vi "test_PhotonPoseEstimator_ClosestToRefPose.vi"(8 "error in (no error)":errorcluster) -> (0 "error out":errorcluster, 3 "Test Passed":bool)   [LabVIEW 2019]
uses:
  <vilib>/Rock Robotics/WPI/ThirdParty/PhotonVisionLib/TypeDef/PhotonEstimatedRobotPoseType.ctl
  <vilib>/Rock Robotics/WPI/ThirdParty/JAS_Junk/TrajLib/TypeDef/POSE3D.ctl
  <vilib>/Rock Robotics/WPI/ThirdParty/JAS_Junk/TrajLib/TypeDef/TRANSLATION3D.ctl
  <vilib>/Rock Robotics/WPI/ThirdParty/JAS_Junk/TrajLib/TypeDef/ROTATION3D.ctl
  <vilib>/Rock Robotics/WPI/ThirdParty/JAS_Junk/TrajLib/TypeDef/QUATERNION.ctl
  <vilib>/Rock Robotics/WPI/ThirdParty/PhotonVisionLib/TypeDef/PhotonTrackedTargetType.ctl
  <vilib>/Rock Robotics/WPI/ThirdParty/PhotonVisionLib/TypeDef/TargetCornerType.ctl
  <vilib>/Rock Robotics/WPI/ThirdParty/JAS_Junk/TrajLib/TypeDef/TRANSFORM3D.ctl
  <vilib>/Rock Robotics/WPI/ThirdParty/PhotonVisionLib/Enum/PhotonPoseStrategy_ENUM.ctl
  <vilib>/Rock Robotics/WPI/ThirdParty/JAS_Junk/TrajLib/VI/Quaternion_New.vi
  <vilib>/Rock Robotics/WPI/ThirdParty/PhotonVisionLib/SubVI/PhotonTargetModel_New_AprilTag36H11.vi
  <vilib>/Rock Robotics/WPI/ThirdParty/JAS_Junk/TrajLib/VI/TimeInterpRotation2d_New.vi
  <vilib>/Rock Robotics/WPI/ThirdParty/PhotonVisionLib/SubVI/PhotonPoseEstimator_Update_All.vi
  <vilib>/Rock Robotics/WPI/ThirdParty/PhotonVisionLib/SubVI/PhotonTargetModel_New_RectPlanar.vi
  <vilib>/Rock Robotics/WPI/ThirdParty/JAS_Junk/TrajLib/Conv_Inches_Meters.vi
  <vilib>/Rock Robotics/WPI/ThirdParty/PhotonVisionLib/SubVI/PhotonPoseEstimator_SetLastPose.vi
  <vilib>/Rock Robotics/WPI/ThirdParty/PhotonVisionLib/SubVI/PhotonPoseEstimator_GetEmptyPose.vi
  <vilib>/Rock Robotics/WPI/ThirdParty/PhotonVisionLib/SubVI/PhotonPoseEstimator_EstimateLowestAmbiguityPose.vi
  <vilib>/Rock Robotics/WPI/ThirdParty/PhotonVisionLib/SubVI/PhotonPoseEstimator_EstimateClosestToCameraHeightPose.vi
  <vilib>/Rock Robotics/WPI/ThirdParty/PhotonVisionLib/SubVI/PhotonPoseEstimator_EstimateClosestToReferencePose.vi
  <vilib>/Rock Robotics/WPI/ThirdParty/PhotonVisionLib/SubVI/PhotonPoseEstimator_GetReferencePose.vi
  <vilib>/Rock Robotics/WPI/ThirdParty/PhotonVisionLib/SubVI/PhotonPoseEstimator_GetLastPose.vi
  <vilib>/Rock Robotics/WPI/ThirdParty/PhotonVisionLib/SubVI/PhotonPoseEstimator_EstimateClosestToLastPose.vi
  <vilib>/Rock Robotics/WPI/ThirdParty/PhotonVisionLib/SubVI/PhotonPoseEstimator_EstimateAverageBestTargetsPose.vi
  <vilib>/Rock Robotics/WPI/ThirdParty/PhotonVisionLib/SubVI/PhotonPoseEstimator_EstimateMultiTagOnCoprocPose.vi
  <vilib>/Rock Robotics/WPI/ThirdParty/PhotonVisionLib/SubVI/PhotonPoseEstimator_EstimatePnpDistanceTrigSolvePose.vi
  <vilib>/Rock Robotics/WPI/ThirdParty/PhotonVisionLib/SubVI/PhotonPoseEstimator_Strategy_constrainedPnpStrategy.vi
  <vilib>/Rock Robotics/WPI/ThirdParty/PhotonVisionLib/SubVI/PhotonPipelineResult_GetTimeStampSecs.vi
  <vilib>/Rock Robotics/WPI/ThirdParty/PhotonVisionLib/SubVI/PhotonTargetModel_New.vi
  <vilib>/Rock Robotics/WPI/ThirdParty/JAS_Junk/TrajLib/VI/Rotation3d_Create_AxisAngle.vi
  <vilib>/Rock Robotics/WPI/ThirdParty/JAS_Junk/TrajLib/VI/Pose3d_New.vi
  <vilib>/Rock Robotics/WPI/ThirdParty/PhotonVisionLib/SubVI/PhotonPipelineResult_HasTargets.vi
  <vilib>/Rock Robotics/WPI/ThirdParty/PhotonVisionLib/SubVI/PhotonPipelineResult_GetTargets.vi
  <vilib>/Rock Robotics/WPI/ThirdParty/PhotonVisionLib/SubVI/PhotonTrackedTarget_GetPoseAmbiguity.vi
  <vilib>/Rock Robotics/WPI/ThirdParty/PhotonVisionLib/SubVI/PhotonTrackedTarget_GetFiducialId.vi
  <vilib>/Rock Robotics/WPI/ThirdParty/PhotonVisionLib/SubVI/PhotonPoseEstimator_GetFieldTags.vi
  <vilib>/Rock Robotics/WPI/ThirdParty/JAS_Junk/TrajLib/VI/AprilTagFieldLayout_GetTagPose.vi
  <vilib>/Rock Robotics/WPI/ThirdParty/JAS_Junk/TrajLib/VI/Pose3d_TransformBy.vi
  <vilib>/Rock Robotics/WPI/ThirdParty/PhotonVisionLib/SubVI/PhotonTrackedTarget_GetBestCameraToTarget.vi
  <vilib>/Rock Robotics/WPI/ThirdParty/JAS_Junk/TrajLib/VI/Transform3d_Inverse.vi
  <vilib>/Rock Robotics/WPI/ThirdParty/PhotonVisionLib/SubVI/PhotonPoseEstimator_GetRobotToCameraTransform.vi
  <vilib>/Rock Robotics/WPI/ThirdParty/PhotonVisionLib/SubVI/PhotonPoseEstimator_GetHighestAmbiguity.vi
  <vilib>/Rock Robotics/WPI/ThirdParty/PhotonVisionLib/SubVI/PhotonEstimatedRobotPose_New.vi
  <vilib>/Rock Robotics/WPI/ThirdParty/PhotonVisionLib/SubVI/PhotonPoseEstimator_Strategy_closestToCameraHeight_calc.vi
  <vilib>/Rock Robotics/WPI/ThirdParty/PhotonVisionLib/SubVI/PhotonTrackedTarget_GetAltCameraToTarget.vi
  <vilib>/Rock Robotics/WPI/ThirdParty/PhotonVisionLib/SubVI/PhotonPoseEstimator_Strategy_closestToReferencePose_calc.vi
  <vilib>/Rock Robotics/WPI/ThirdParty/PhotonVisionLib/SubVI/PhotonPoseEstimator_Strategy_averageBestTargets_calc.vi
  <vilib>/Rock Robotics/WPI/ThirdParty/JAS_Junk/TrajLib/VI/Rotation3d_Plus.vi
  <vilib>/Rock Robotics/WPI/ThirdParty/JAS_Junk/TrajLib/VI/Translation3d_Plus.vi
  <vilib>/Rock Robotics/WPI/ThirdParty/JAS_Junk/TrajLib/VI/Translation3d_Times.vi
  <vilib>/Rock Robotics/WPI/ThirdParty/JAS_Junk/TrajLib/VI/Rotation3d_Times.vi
  <vilib>/Rock Robotics/WPI/ThirdParty/JAS_Junk/TrajLib/VI/Rotation3d_Create_Default.vi
  <vilib>/Rock Robotics/WPI/ThirdParty/JAS_Junk/TrajLib/VI/Translation3d_Create_Default.vi
  <vilib>/Rock Robotics/WPI/ThirdParty/JAS_Junk/TrajLib/VI/Pose3d_New_Default.vi
  <vilib>/Rock Robotics/WPI/ThirdParty/JAS_Junk/TrajLib/VI/Pose3d_Plus.vi
  <vilib>/Rock Robotics/WPI/ThirdParty/JAS_Junk/TrajLib/VI/Pose3d_RelativeTo.vi
  <vilib>/Rock Robotics/WPI/ThirdParty/JAS_Junk/TrajLib/VI/AprilTagFieldLayout_GetOriginPosition.vi
  <vilib>/Rock Robotics/WPI/ThirdParty/PhotonVisionLib/SubVI/PhotonPipelineResult_GetMultiTagResult.vi
  <vilib>/Rock Robotics/WPI/ThirdParty/PhotonVisionLib/SubVI/PhotonPipelineResult_GetBestTarget.vi
  <vilib>/Rock Robotics/WPI/ThirdParty/PhotonVisionLib/SubVI/PhotonTrackedTarget_GetPitch.vi
  <vilib>/Rock Robotics/WPI/ThirdParty/PhotonVisionLib/SubVI/PhotonTrackedTarget_GetYaw.vi
  <vilib>/Rock Robotics/WPI/ThirdParty/JAS_Junk/TrajLib/Units_DegreesToRadians.vi
  <vilib>/Rock Robotics/WPI/ThirdParty/JAS_Junk/TrajLib/VI/Transform3d_GetTranslation3d.vi
  <vilib>/Rock Robotics/WPI/ThirdParty/JAS_Junk/TrajLib/VI/Translation3d_GetNorm.vi
  <vilib>/Rock Robotics/WPI/ThirdParty/JAS_Junk/TrajLib/VI/Translation3d_Create_DistAng.vi
  <vilib>/Rock Robotics/WPI/ThirdParty/JAS_Junk/TrajLib/VI/Translation3d_RotateBy.vi
  <vilib>/Rock Robotics/WPI/ThirdParty/JAS_Junk/TrajLib/VI/Translation3d_ToTranslation2d.vi
  <vilib>/Rock Robotics/WPI/ThirdParty/JAS_Junk/TrajLib/Translation2d_RotateBy.vi
  <vilib>/Rock Robotics/WPI/ThirdParty/JAS_Junk/TrajLib/VI/Transform3d_GetRotation3d.vi
  <vilib>/Rock Robotics/WPI/ThirdParty/JAS_Junk/TrajLib/VI/Pose3d_ToPose2d.vi
  <vilib>/Rock Robotics/WPI/ThirdParty/JAS_Junk/TrajLib/Pose2d_getTranslation.vi
  <vilib>/Rock Robotics/WPI/ThirdParty/JAS_Junk/TrajLib/Translation2d_Plus.vi
  <vilib>/Rock Robotics/WPI/ThirdParty/JAS_Junk/TrajLib/Translation2d_UnaryMinus.vi
  <vilib>/Rock Robotics/WPI/ThirdParty/JAS_Junk/TrajLib/Pose2d_New_TRRO.vi
  <vilib>/Rock Robotics/WPI/ThirdParty/JAS_Junk/TrajLib/VI/Pose3d_New_Pose2d.vi
  <vilib>/Rock Robotics/WPI/ThirdParty/JAS_Junk/TrajLib/VI/TimeInterpRotation2d_GetSample.vi
  <vilib>/Rock Robotics/WPI/ThirdParty/PhotonVisionLib/SubVI/PhotonPoseEstimator_GetHeadingBuffer.vi
  <vilib>/Rock Robotics/WPI/ThirdParty/JAS_Junk/TrajLib/VI/Vector_Norm.vi
  <vilib>/Rock Robotics/WPI/ThirdParty/JAS_Junk/TrajLib/VecBuilder_ArrayBy1Fill.vi
  <vilib>/Rock Robotics/WPI/ThirdParty/JAS_Junk/TrajLib/VI/AprilTag_GetAll.vi
  <vilib>/Rock Robotics/WPI/ThirdParty/JAS_Junk/TrajLib/VI/Pose3d_getTranslation3d.vi
  <vilib>/Rock Robotics/WPI/ThirdParty/JAS_Junk/TrajLib/VI/Pose3d_getRotation3d.vi
  <vilib>/Rock Robotics/WPI/ThirdParty/JAS_Junk/TrajLib/VI/Rotation3d_ToRotation2d.vi
  <vilib>/Rock Robotics/WPI/ThirdParty/JAS_Junk/TrajLib/Transform2d_Create_TransRot.vi
  <vilib>/Rock Robotics/WPI/ThirdParty/JAS_Junk/TrajLib/VI/Rotation3d_UnaryMinus.vi
  <vilib>/Rock Robotics/WPI/ThirdParty/JAS_Junk/TrajLib/VI/Translation3d_UnaryMinus.vi
  <vilib>/Rock Robotics/WPI/ThirdParty/JAS_Junk/TrajLib/VI/Transform3d_GetXYZ.vi
  <vilib>/Rock Robotics/WPI/ThirdParty/JAS_Junk/TrajLib/VI/Pose3d_getXYZ.vi
  <vilib>/Rock Robotics/WPI/ThirdParty/PhotonVisionLib/SubVI/PhotonPoseEstimator_CalcDifference.vi
  <vilib>/Rock Robotics/WPI/ThirdParty/JAS_Junk/TrajLib/VI/Rotation3d_RotateBy.vi
  <vilib>/Rock Robotics/WPI/ThirdParty/JAS_Junk/TrajLib/VI/Translation3d_GetXYZ.vi
  <vilib>/Rock Robotics/WPI/ThirdParty/JAS_Junk/TrajLib/VI/Rotation3d_GetQuaterion.vi
  <vilib>/Rock Robotics/WPI/ThirdParty/JAS_Junk/TrajLib/VI/Quaternion_Get_Vect.vi
  <vilib>/Rock Robotics/WPI/ThirdParty/JAS_Junk/TrajLib/VI/Quaternion_Get_W.vi
  <vilib>/Rock Robotics/WPI/ThirdParty/JAS_Junk/TrajLib/VI/Quaternion_New_Default.vi
  <vilib>/Rock Robotics/WPI/ThirdParty/JAS_Junk/TrajLib/VI/Transform3d_Create_Pose3dPose3d.vi
  <vilib>/Rock Robotics/WPI/ThirdParty/JAS_Junk/TrajLib/Conv_Deg_Radians.vi
  <vilib>/Rock Robotics/WPI/ThirdParty/JAS_Junk/TrajLib/VI/Quaternion_Times.vi
  <vilib>/Rock Robotics/WPI/ThirdParty/JAS_Junk/TrajLib/VI/Quaternion_Inverse.vi
  <vilib>/Rock Robotics/WPI/ThirdParty/JAS_Junk/TrajLib/VI/Quaternion_Get_All.vi
  <vilib>/Rock Robotics/WPI/ThirdParty/JAS_Junk/TrajLib/Translation2d_Create.vi
  <vilib>/Rock Robotics/WPI/ThirdParty/JAS_Junk/TrajLib/Pose2d_getXYAngle.vi
  <vilib>/Rock Robotics/WPI/ThirdParty/JAS_Junk/TrajLib/Rotation2d_Interpolate.vi
  <vilib>/Rock Robotics/WPI/ThirdParty/JAS_Junk/TrajLib/MatBuilder_Create.vi
  <vilib>/Rock Robotics/WPI/ThirdParty/JAS_Junk/TrajLib/Rotation2d_CreateAngle.vi
  <vilib>/Rock Robotics/WPI/ThirdParty/JAS_Junk/TrajLib/VI/Rotation3d_GetXYZ.vi
  <vilib>/Rock Robotics/WPI/ThirdParty/JAS_Junk/TrajLib/VI/Rotation3d_Create_Quaternion.vi
  <vilib>/Rock Robotics/WPI/ThirdParty/JAS_Junk/TrajLib/VI/Translation3d_GetDistance.vi
  <vilib>/Rock Robotics/WPI/ThirdParty/JAS_Junk/TrajLib/VI/Translation3d_Minus.vi
  <vilib>/Rock Robotics/WPI/ThirdParty/JAS_Junk/TrajLib/VI/Rotation3d_Minus.vi
  <vilib>/Rock Robotics/WPI/ThirdParty/JAS_Junk/TrajLib/Rotation2d_Plus.vi
  <vilib>/Rock Robotics/WPI/ThirdParty/JAS_Junk/TrajLib/Rotation2d_Minus.vi
  <vilib>/Rock Robotics/WPI/ThirdParty/JAS_Junk/TrajLib/MathUtil_Clamp.vi
  <vilib>/Rock Robotics/WPI/ThirdParty/JAS_Junk/TrajLib/Rotation2d_Times.vi
  <vilib>/Rock Robotics/WPI/ThirdParty/JAS_Junk/TrajLib/VI/Quaternion_Normalize.vi
  <vilib>/Rock Robotics/WPI/ThirdParty/JAS_Junk/TrajLib/Rotation2d_RotateBy.vi
  <vilib>/Rock Robotics/WPI/ThirdParty/JAS_Junk/TrajLib/Rotation2d_UnaryMinus.vi
  <vilib>/Rock Robotics/WPI/ThirdParty/JAS_Junk/TrajLib/Rotation2d_CreateXY.vi
  <vilib>/Rock Robotics/WPI/ThirdParty/JAS_Junk/TrajLib/Util_CalcDist.vi
  <vilib>/Rock Robotics/WPI/ThirdParty/PhotonVisionLib/SubVI/PhotonVision_Globals.vi
  <vilib>/gmath/interp.llb/Search Ordered Table.vi
  <vilib>/Rock Robotics/WPI/ThirdParty/JAS_Junk/TrajLib/Trajectory_Library.lvlib
  <vilib>/Rock Robotics/WPI/ThirdParty/PhotonVisionLib/PhotonVisionLib.lvlib
panel:
  out "Test 2 Passed":bool
  out "Test 1 Passed":bool
  out "Pos Found":bool
  out "PhotonEstimatedRobotPose":T1={"EstimatedPose"={"Translation3d"={"X"=0.0, "Y"=0.0, "Z"=0.0}, "Rotation3d"={"Q_quaternion"={"R"=1.0, "V"=[0.0, 0.0, 0.0]}}}, "TimeStamp_Seconds"=0.0, "targetsUsed"=[], "Strategy"=enum."LOWEST_AMBIGUITY"} {"targetsUsed"."AltCameraToTarget"."TRANSLATION3D"."Z" format="%14.3f"; "targetsUsed"."AltCameraToTarget"."TRANSLATION3D"."Y" format="%14.3f"; "targetsUsed"."AltCameraToTarget"."TRANSLATION3D"."X" format="%14.3f"; "targetsUsed"."BestCameraToTarget"."TRANSLATION3D"."Z" format="%14.3f"; "targetsUsed"."BestCameraToTarget"."TRANSLATION3D"."Y" format="%14.3f"; "targetsUsed"."BestCameraToTarget"."TRANSLATION3D"."X" format="%14.3f"; "EstimatedPose"."Translation3d"."Z" format="%14.3f"; "EstimatedPose"."Translation3d"."Y" format="%14.3f"; "EstimatedPose"."Translation3d"."X" format="%14.3f"}
  out "Test 0 Passed":bool
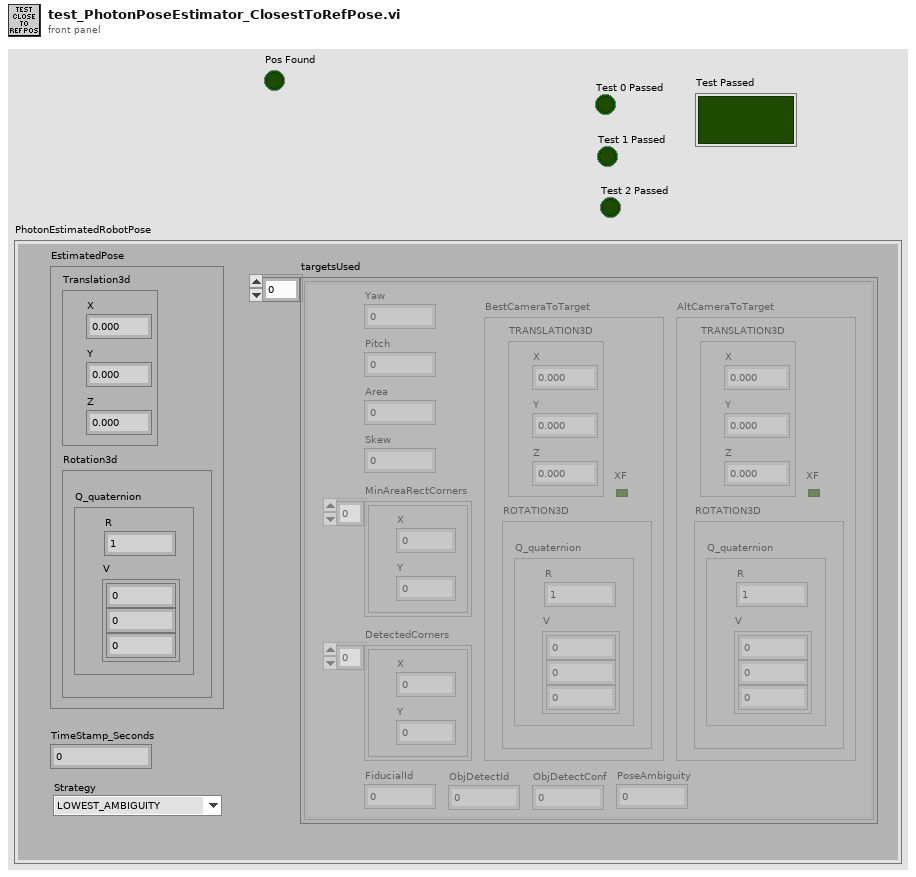
[diagram p1: front panel]
types:
  T1 = typedef "PhotonVisionLib.lvlib/PhotonEstimatedRobotPoseType.ctl" = cluster{"EstimatedPose":T2, "TimeStamp_Seconds":dbl, "targetsUsed":T6[], "Strategy":T9}
  T2 = typedef "Trajectory_Library.lvlib/POSE3D.ctl" = cluster{"Translation3d":T3, "Rotation3d":T4}
  T3 = typedef "Trajectory_Library.lvlib/TRANSLATION3D.ctl" = cluster{"X":dbl, "Y":dbl, "Z":dbl}
  T4 = typedef "Trajectory_Library.lvlib/ROTATION3D.ctl" = cluster{"Q_quaternion":T5}
  T5 = typedef "Trajectory_Library.lvlib/QUATERNION.ctl" = cluster{"R":dbl, "V":dbl[]}
  T6 = typedef "PhotonVisionLib.lvlib/PhotonTrackedTargetType.ctl" = cluster{"Yaw":dbl, "Pitch":dbl, "Area":dbl, "Skew":dbl, "MinAreaRectCorners":T7[], "BestCameraToTarget":T8, "FiducialId":i32, "AltCameraToTarget":T8, "PoseAmbiguity":dbl, "DetectedCorners":T7[], "ObjDetectId":i32, "ObjDetectConf":sgl}
  T7 = typedef "PhotonVisionLib.lvlib/TargetCornerType.ctl" = cluster{"X":dbl, "Y":dbl}
  T8 = typedef "Trajectory_Library.lvlib/TRANSFORM3D.ctl" = cluster{"TRANSLATION3D":T3, "ROTATION3D":T4, "XF":bool}
  T9 = typedef "PhotonVisionLib.lvlib/PhotonPoseStrategy_ENUM.ctl" = enum16{"LOWEST_AMBIGUITY", "CLOSEST_TO_CAMERA_HEIGHT", "CLOSEST_TO_REFERENCE_POSE", "CLOSEST_TO_LAST_POSE", "AVERAGE_BEST_TARGETS", "MULTI_TAG_PNP_ON_COPROCESSOR", "MULTI_TAG_PNP_ON_RIO", "PNP_DISTANCE_TRIG_SOLVE", "CONSTRAINED_SOLVEPNP"}
  T10 = typedef "Trajectory_Library.lvlib/AprilTagFieldLayout.ctl" = cluster{"AprilTagMap":map{i32, T11}, "FieldLength":dbl, "FieldWidth":dbl, "OriginPosition ":T12, "OriginPose3d":T2}
  T11 = typedef "Trajectory_Library.lvlib/AprilTag.ctl" = cluster{"ID":i32, "POSE3D":T2}
  T12 = typedef "Trajectory_Library.lvlib/AprilTagFieldLayoutOrignPosition_ENUM.ctl" = enum16{"kBlueAllianceWallRightSide,", "kRedAllianceWallRightSide,"}
  T13 = typedef "PhotonVisionLib.lvlib/PhotonPipelineMetadataType.ctl" = cluster{"CaptureTimestampMicros":i64, "PublishTimestampMicros":i64, "SequenceID":i64, "TimeSinceLastPong":i64}
  T14 = typedef "PhotonVisionLib.lvlib/PhotonPipelineResultType.ctl" = cluster{"Targets":T6[], "PhotonMultiTargetPNPResult":T15, "PhotonPipelineMetadata":T13}
  T15 = typedef "PhotonVisionLib.lvlib/PhotonMultiTargetPNPResultType.ctl" = cluster{"PhotonPNPResult":T16, "FiducialIDsUsed":i16[]}
  T16 = typedef "PhotonVisionLib.lvlib/PhotonPNPResultType.ctl" = cluster{"IsPresent":bool, "bestReprojErr":dbl, "altReprojErr":dbl, "ambiguity":dbl, "Best":T8, "Alt":T8}
  T17 = typedef "PhotonVisionLib.lvlib/PhotonPoseEstimatorType.ctl" = cluster{"LastPose":T2, "ReferencePose":T2, "FieldTags":T10, "PrimaryStratety":T9, "Camera":string, "RobotToCamera":T8, "ReportedErrors":dbl[], "HighestAmbiguity":dbl, "MultiTagFallbackStrategy":T9, "PoseCacheTimeoutSec":dbl, "PhotonTargetModel":T18, "BaseNTName":string}
  T18 = typedef "PhotonVisionLib.lvlib/PhotonTargetModel.ctl" = cluster{"Vertices":T3[], "IsPlaner":bool, "IsSpherical":bool}
  T19 = typedef "PhotonVisionLib.lvlib/PhotonPoseEstimator_Configuration.ctl" = cluster{"Primary Strategy":T9, "Camera":string, "Initial Pose":T2, "HighestAmbiguity":dbl, "RobotToCamera":T8, "FallBack Strategy":T9, "BaseNTName":string}
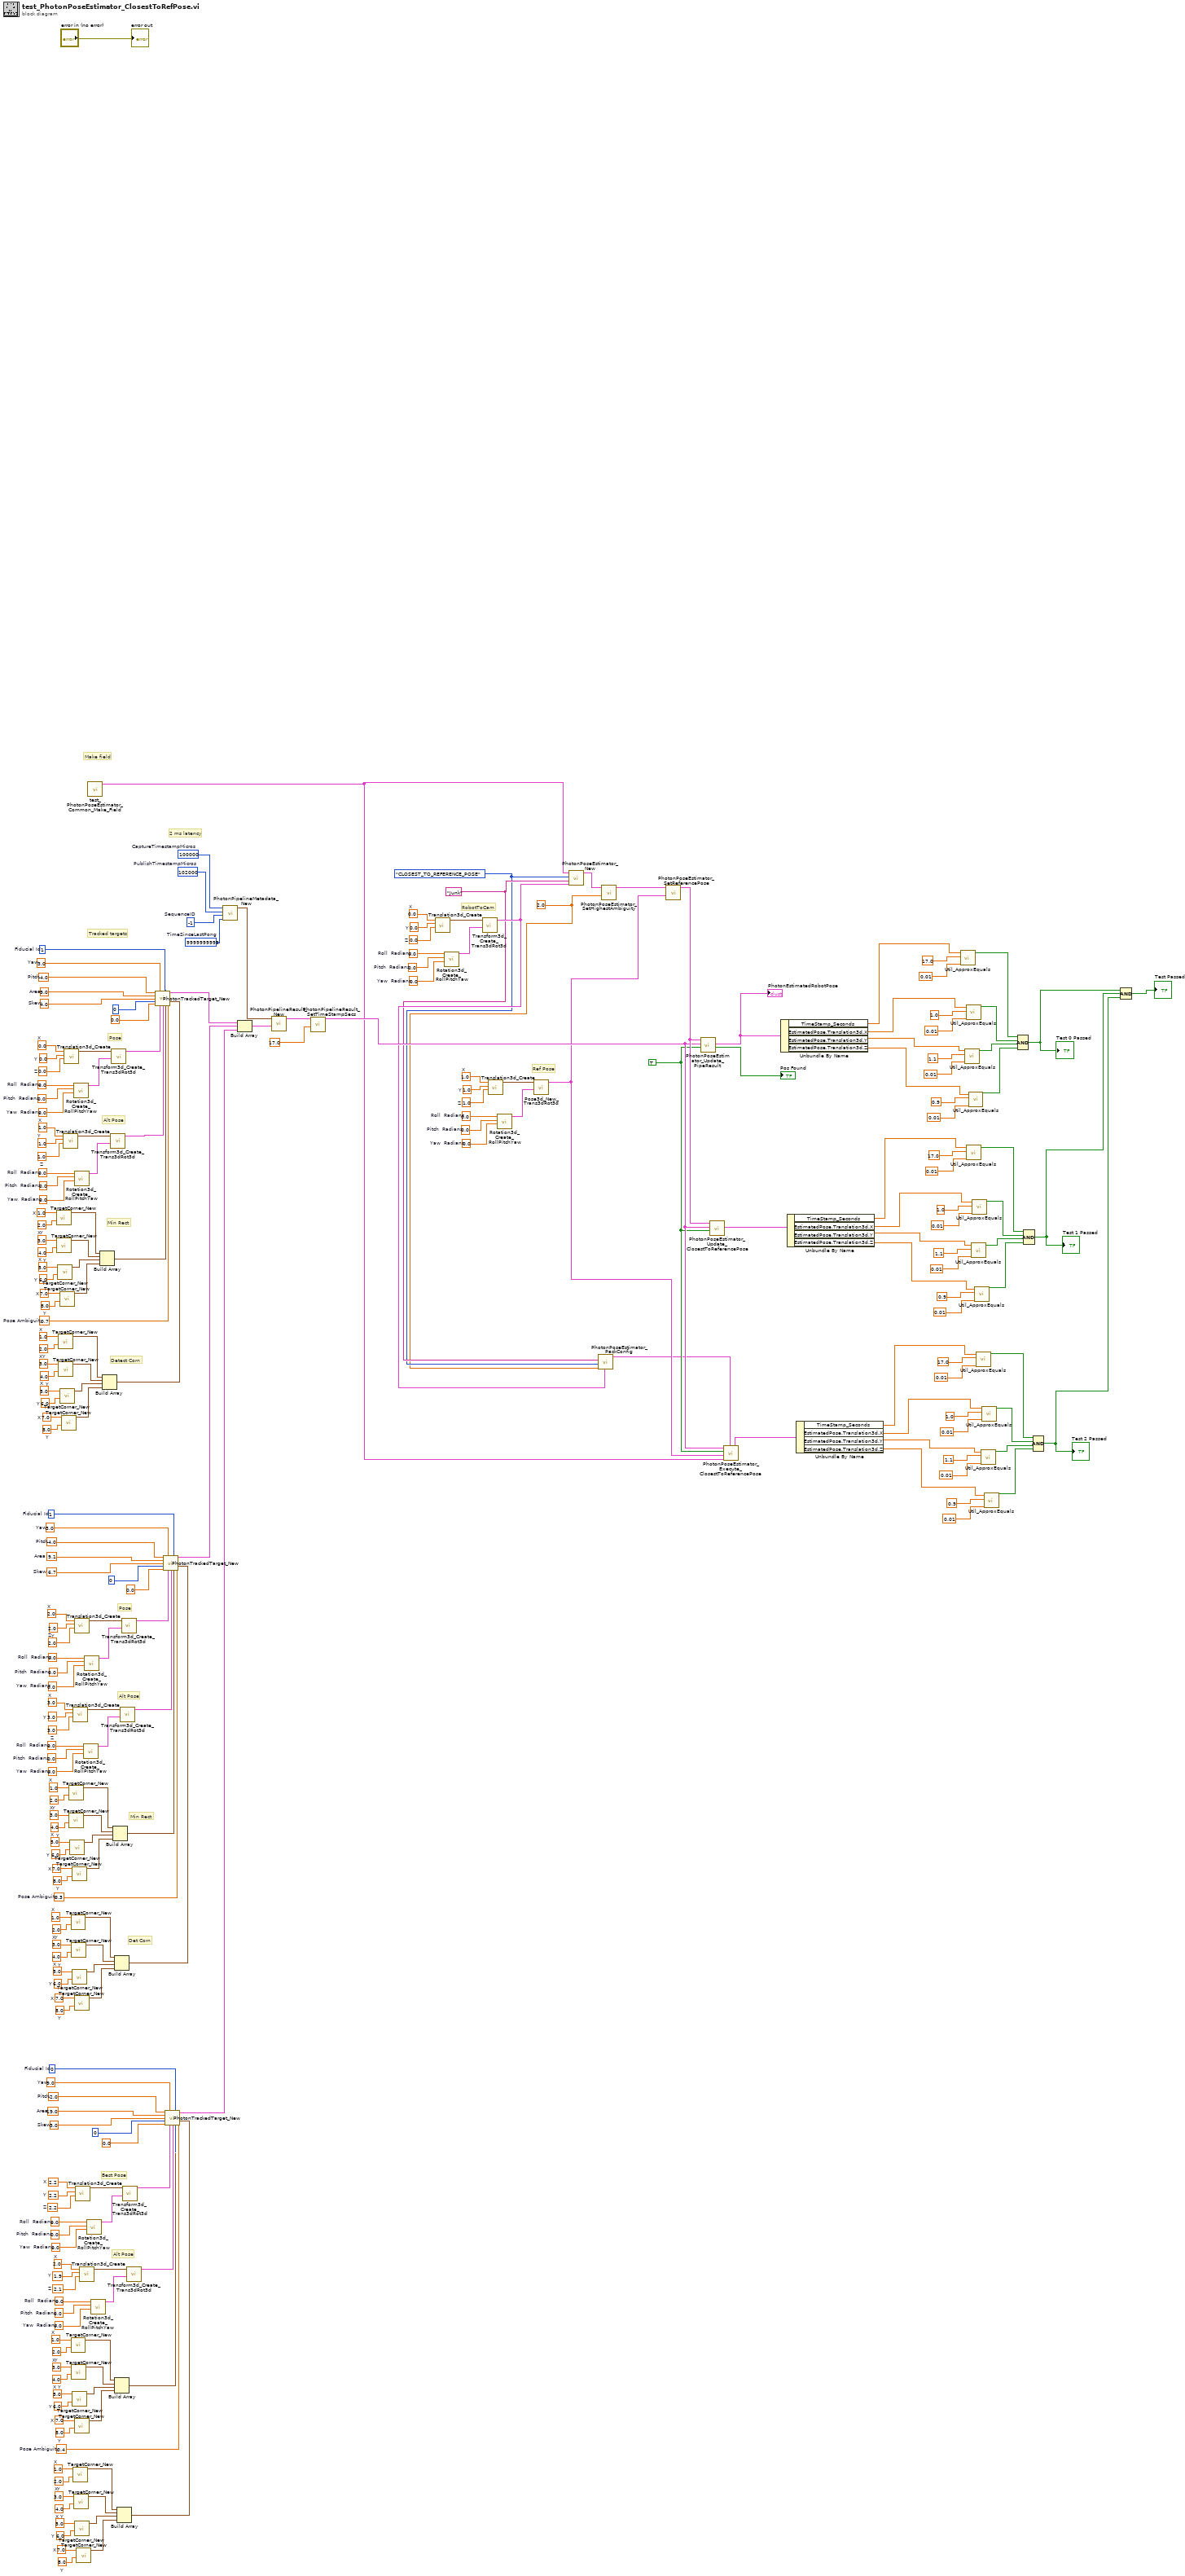
[diagram p0: block diagram]
diagram:
  w1 = 2.0 ("HighestAmbiguity")
  w56 = i64 100000  # CaptureTimestampMicros
  w57 = i64 102000  # PublishTimestampMicros
  w58 = i64 -1  # SequenceID
  w59 = i64 9999999999  # TimeSinceLastPong
  w8 = TRUE ("Has Results")
  w66 = 0.0  # Roll  Radians
  w65 = 0.0  # Pitch  Radians
  w64 = 0.0  # Yaw  Radians
  w69 = 1.0  # Z
  w68 = 1.0  # X
  w67 = 1.0  # Y
  w78 = 0.0  # Roll  Radians
  w77 = 0.0  # Pitch  Radians
  w76 = 0.0  # Yaw  Radians
  w81 = 0.0  # Z
  w80 = 0.0  # X
  w79 = 0.0  # Y
  w3 = "Junk" ("Camera")
  w2 = PhotonPoseStrategy_ENUM."CLOSEST_TO_REFERENCE_POSE" ("Strategy")
  w103 = 0.0  # Roll  Radians
  w102 = 0.0  # Pitch  Radians
  w101 = 0.0  # Yaw  Radians
  w106 = 2.2  # Z
  w105 = 2.2  # X
  w104 = 2.2  # Y
  w111 = 0.0  # Roll  Radians
  w110 = 0.0  # Pitch  Radians
  w109 = 0.0  # Yaw  Radians
  w114 = 2.1  # Z
  w113 = 2.0  # X
  w112 = 1.9  # Y
  w121 = 7.0  # X
  w122 = 8.0  # Y
  w123 = 5.0  # X
  w124 = 6.0  # Y
  w125 = 3.0  # X
  w126 = 4.0  # Y
  w127 = 1.0  # X
  w128 = 2.0  # Y
  w133 = 7.0  # X
  w134 = 8.0  # Y
  w135 = 5.0  # X
  w136 = 6.0  # Y
  w137 = 3.0  # X
  w138 = 4.0  # Y
  w139 = 1.0  # X
  w140 = 2.0  # Y
  w141 = -2.0  # Pitch
  w142 = 19.0  # Area
  w143 = 3.0  # Skew
  w144 = 0  # Fiducial Id
  w145 = 0.4  # Pose Ambiguity
  w146 = 9.0  # Yaw
  w153 = 0.0  # Roll  Radians
  w152 = 0.0  # Pitch  Radians
  w151 = 0.0  # Yaw  Radians
  w156 = 2.0  # Z
  w155 = 2.0  # X
  w154 = 2.0  # Y
  w161 = 0.0  # Roll  Radians
  w160 = 0.0  # Pitch  Radians
  w159 = 0.0  # Yaw  Radians
  w164 = 3.0  # Z
  w163 = 3.0  # X
  w162 = 3.0  # Y
  w171 = 7.0  # X
  w172 = 8.0  # Y
  w173 = 5.0  # X
  w174 = 6.0  # Y
  w175 = 3.0  # X
  w176 = 4.0  # Y
  w177 = 1.0  # X
  w178 = 2.0  # Y
  w183 = 7.0  # X
  w184 = 8.0  # Y
  w185 = 5.0  # X
  w186 = 6.0  # Y
  w187 = 3.0  # X
  w188 = 4.0  # Y
  w189 = 1.0  # X
  w190 = 2.0  # Y
  w191 = -4.0  # Pitch
  w192 = 9.1  # Area
  w193 = 6.7  # Skew
  w194 = 1  # Fiducial Id
  w195 = 0.3  # Pose Ambiguity
  w196 = 3.0  # Yaw
  w203 = 0.0  # Roll  Radians
  w202 = 0.0  # Pitch  Radians
  w201 = 0.0  # Yaw  Radians
  w206 = 0.0  # Z
  w205 = 0.0  # X
  w204 = 0.0  # Y
  w211 = 0.0  # Roll  Radians
  w210 = 0.0  # Pitch  Radians
  w209 = 0.0  # Yaw  Radians
  w214 = 1.0  # Z
  w213 = 1.0  # X
  w212 = 1.0  # Y
  w221 = 7.0  # X
  w222 = 8.0  # Y
  w223 = 5.0  # X
  w224 = 6.0  # Y
  w225 = 3.0  # X
  w226 = 4.0  # Y
  w227 = 1.0  # X
  w228 = 2.0  # Y
  w233 = 7.0  # X
  w234 = 8.0  # Y
  w235 = 5.0  # X
  w236 = 6.0  # Y
  w237 = 3.0  # X
  w238 = 4.0  # Y
  w239 = 1.0  # X
  w240 = 2.0  # Y
  w241 = -4.0  # Pitch
  w242 = 9.0  # Area
  w243 = 4.0  # Skew
  w244 = 1  # Fiducial Id
  w245 = 0.7  # Pose Ambiguity
  w246 = 3.0  # Yaw
  # "2 ms latency"
  # "Ref Pose"
  # "RobotToCam"
  # "Det Corn"
  # "Min Rect"
  # "Pose"
  # "Detect Corn"
  # "Min Rect"
  # "Tracked targets"
  # "Make field"
  # "Best Pose"
  # "Alt Pose"
  # "Alt Pose"
  # "Pose"
  # "Alt Pose"
  n1 = call <vilib>:"TargetCorner_New.vi"("Y"=w240, "X"=w239) -> ("TargetCorner"=w232:T7)  [unwired: 9 in]
  n2 = call <vilib>:"TargetCorner_New.vi"("Y"=w238, "X"=w237) -> ("TargetCorner"=w231:T7)  [unwired: 9 in]
  n3 = call <vilib>:"TargetCorner_New.vi"("Y"=w236, "X"=w235) -> ("TargetCorner"=w230:T7)  [unwired: 9 in]
  n4 = call <vilib>:"TargetCorner_New.vi"("Y"=w228, "X"=w227) -> ("TargetCorner"=w220:T7)  [unwired: 9 in]
  n5 = call <vilib>:"TargetCorner_New.vi"("Y"=w226, "X"=w225) -> ("TargetCorner"=w219:T7)  [unwired: 9 in]
  n6 = call <vilib>:"TargetCorner_New.vi"("Y"=w234, "X"=w233) -> ("TargetCorner"=w229:T7)  [unwired: 9 in]
  n7 = call <vilib>:"TargetCorner_New.vi"("Y"=w224, "X"=w223) -> ("TargetCorner"=w218:T7)  [unwired: 9 in]
  n8 = call <vilib>:"TargetCorner_New.vi"("Y"=w222, "X"=w221) -> ("TargetCorner"=w217:T7)  [unwired: 9 in]
  n9 = call <vilib>:"Translation3d_Create.vi"("Z"=w214, "Y"=w212, "X"=w213) -> ("TRANSLATION3D"=w208:T3)  [unwired: 8 in]
  n10 = call <vilib>:"Translation3d_Create.vi"("Z"=w206, "Y"=w204, "X"=w205) -> ("TRANSLATION3D"=w200:T3)  [unwired: 8 in]
  n11 = call <vilib>:"TargetCorner_New.vi"("Y"=w190, "X"=w189) -> ("TargetCorner"=w182:T7)  [unwired: 9 in]
  n12 = call <vilib>:"TargetCorner_New.vi"("Y"=w188, "X"=w187) -> ("TargetCorner"=w181:T7)  [unwired: 9 in]
  n13 = call <vilib>:"TargetCorner_New.vi"("Y"=w186, "X"=w185) -> ("TargetCorner"=w180:T7)  [unwired: 9 in]
  n14 = call <vilib>:"TargetCorner_New.vi"("Y"=w178, "X"=w177) -> ("TargetCorner"=w170:T7)  [unwired: 9 in]
  n15 = call <vilib>:"TargetCorner_New.vi"("Y"=w140, "X"=w139) -> ("TargetCorner"=w132:T7)  [unwired: 9 in]
  n16 = call <vilib>:"TargetCorner_New.vi"("Y"=w176, "X"=w175) -> ("TargetCorner"=w169:T7)  [unwired: 9 in]
  n17 = call <vilib>:"TargetCorner_New.vi"("Y"=w138, "X"=w137) -> ("TargetCorner"=w131:T7)  [unwired: 9 in]
  n18 = call <vilib>:"TargetCorner_New.vi"("Y"=w184, "X"=w183) -> ("TargetCorner"=w179:T7)  [unwired: 9 in]
  n19 = call <vilib>:"TargetCorner_New.vi"("Y"=w174, "X"=w173) -> ("TargetCorner"=w168:T7)  [unwired: 9 in]
  n20 = call <vilib>:"TargetCorner_New.vi"("Y"=w136, "X"=w135) -> ("TargetCorner"=w130:T7)  [unwired: 9 in]
  n21 = call <vilib>:"Translation3d_Create.vi"("Z"=w164, "Y"=w162, "X"=w163) -> ("TRANSLATION3D"=w158:T3)  [unwired: 8 in]
  n22 = call <vilib>:"TargetCorner_New.vi"("Y"=w128, "X"=w127) -> ("TargetCorner"=w120:T7)  [unwired: 9 in]
  n23 = call <vilib>:"Rotation3d_Create_RollPitchYaw.vi"("Yaw"=w201, "Pitch"=w202, "Roll"=w203) -> ("Rotation3d"=w199:T4)  [unwired: 8 in]
  n24 = call <vilib>:"TargetCorner_New.vi"("Y"=w126, "X"=w125) -> ("TargetCorner"=w119:T7)  [unwired: 9 in]
  n25 = call <vilib>:"Rotation3d_Create_RollPitchYaw.vi"("Yaw"=w209, "Pitch"=w210, "Roll"=w211) -> ("Rotation3d"=w207:T4)  [unwired: 8 in]
  n26 = call <vilib>:"Translation3d_Create.vi"("Z"=w156, "Y"=w154, "X"=w155) -> ("TRANSLATION3D"=w150:T3)  [unwired: 8 in]
  n27 = call <vilib>:"TargetCorner_New.vi"("Y"=w172, "X"=w171) -> ("TargetCorner"=w167:T7)  [unwired: 9 in]
  n28 = call <vilib>:"TargetCorner_New.vi"("Y"=w134, "X"=w133) -> ("TargetCorner"=w129:T7)  [unwired: 9 in]
  n29 = call <vilib>:"TargetCorner_New.vi"("Y"=w124, "X"=w123) -> ("TargetCorner"=w118:T7)  [unwired: 9 in]
  n30 = call <vilib>:"Translation3d_Create.vi"("Z"=w106, "Y"=w104, "X"=w105) -> ("TRANSLATION3D"=w100:T3)  [unwired: 8 in]
  n31 = call <vilib>:"TargetCorner_New.vi"("Y"=w122, "X"=w121) -> ("TargetCorner"=w117:T7)  [unwired: 9 in]
  n32 = call <vilib>:"Translation3d_Create.vi"("Z"=w114, "Y"=w112, "X"=w113) -> ("TRANSLATION3D"=w108:T3)  [unwired: 8 in]
  n33 = call <vilib>:"Rotation3d_Create_RollPitchYaw.vi"("Yaw"=w159, "Pitch"=w160, "Roll"=w161) -> ("Rotation3d"=w157:T4)  [unwired: 8 in]
  n34 = call <vilib>:"Rotation3d_Create_RollPitchYaw.vi"("Yaw"=w151, "Pitch"=w152, "Roll"=w153) -> ("Rotation3d"=w149:T4)  [unwired: 8 in]
  n35 = call <vilib>:"Rotation3d_Create_RollPitchYaw.vi"("Yaw"=w101, "Pitch"=w102, "Roll"=w103) -> ("Rotation3d"=w99:T4)  [unwired: 8 in]
  n36 = call "test_PhotonPoseEstimator_Common_Make_Field.vi"() -> ("AprilTagFieldLayout"=w6:T10)  [unwired: 11 in]
  n37 = call <vilib>:"Rotation3d_Create_RollPitchYaw.vi"("Yaw"=w109, "Pitch"=w110, "Roll"=w111) -> ("Rotation3d"=w107:T4)  [unwired: 8 in]
  n38 = Build Array(w232, w231, w230, w229) -> (w216:T7[])
  n39 = Build Array(w220, w219, w218, w217) -> (w215:T7[])
  n40 = call <vilib>:"Transform3d_Create_Trans3dRot3d.vi"("Rotation3d"=w207, "Translation3d"=w208) -> ("Transform3d"=w197:T8)  [unwired: 9 in]
  n41 = call <vilib>:"Transform3d_Create_Trans3dRot3d.vi"("Rotation3d"=w199, "Translation3d"=w200) -> ("Transform3d"=w198:T8)  [unwired: 9 in]
  n42 = Build Array(w182, w181, w180, w179) -> (w166:T7[])
  n43 = Build Array(w170, w169, w168, w167) -> (w165:T7[])
  n44 = Build Array(w132, w131, w130, w129) -> (w116:T7[])
  n45 = Build Array(w120, w119, w118, w117) -> (w115:T7[])
  n46 = call <vilib>:"Transform3d_Create_Trans3dRot3d.vi"("Rotation3d"=w157, "Translation3d"=w158) -> ("Transform3d"=w147:T8)  [unwired: 9 in]
  n47 = call <vilib>:"Transform3d_Create_Trans3dRot3d.vi"("Rotation3d"=w149, "Translation3d"=w150) -> ("Transform3d"=w148:T8)  [unwired: 9 in]
  n48 = call <vilib>:"Transform3d_Create_Trans3dRot3d.vi"("Rotation3d"=w99, "Translation3d"=w100) -> ("Transform3d"=w98:T8)  [unwired: 9 in]
  n49 = call <vilib>:"Transform3d_Create_Trans3dRot3d.vi"("Rotation3d"=w107, "Translation3d"=w108) -> ("Transform3d"=w97:T8)  [unwired: 9 in]
  n50 = call <vilib>:"PhotonTrackedTarget_New.vi"("Pitch"=w241, "Yaw"=w246, "Fiducial Id"=w244, "Area"=w242, "Skew"=w243, "ObjDetectId"=0, "DetectedCorners"=w215, "DetectObjConf"=sgl 0.0, "BestCameraToTarget"=w198, "AltCameraToTarget"=w197, "MinAreaRectCorners"=w216, "Pose Ambiguity"=w245) -> ("TrackedTarget"=w96:T6)  [unwired: 3 in]
  n51 = call <vilib>:"PhotonTrackedTarget_New.vi"("Pitch"=w191, "Yaw"=w196, "Fiducial Id"=w194, "Area"=w192, "Skew"=w193, "ObjDetectId"=0, "DetectedCorners"=w165, "DetectObjConf"=sgl 0.0, "BestCameraToTarget"=w148, "AltCameraToTarget"=w147, "MinAreaRectCorners"=w166, "Pose Ambiguity"=w195) -> ("TrackedTarget"=w95:T6)  [unwired: 3 in]
  n52 = call <vilib>:"PhotonTrackedTarget_New.vi"("Pitch"=w141, "Yaw"=w146, "Fiducial Id"=w144, "Area"=w142, "Skew"=w143, "ObjDetectId"=0, "DetectedCorners"=w115, "DetectObjConf"=sgl 0.0, "BestCameraToTarget"=w98, "AltCameraToTarget"=w97, "MinAreaRectCorners"=w116, "Pose Ambiguity"=w145) -> ("TrackedTarget"=w94:T6)  [unwired: 3 in]
  n53 = call <vilib>:"PhotonPipelineMetadata_New.vi"("TimeSinceLastPong"=w59, "SequenceID"=w58, "PublishTimestampMicros"=w57, "CaptureTimestampMicros"=w56) -> ("PhotonPipelineMetadata"=w55:T13)  [unwired: 7 in]
  n54 = Build Array(w96, w95, w94) -> (w93:T6[])
  n55 = call <vilib>:"PhotonPipelineResult_New.vi"("TrackedTargets"=w93, "Metadata"=w55) -> ("PhotonPipelineResult"=w92:T14)  [unwired: 9 in]
  n56 = call <vilib>:"PhotonPipelineResult_SetTimeStampSecs.vi"("TimeStampSec"=17.0, "PhotonPipelineResult"=w92) -> ("Out PhotonPipelineResult"=w9:T14)  [unwired: 9 in]
  n57 = call <vilib>:"Translation3d_Create.vi"("Z"=w81, "Y"=w79, "X"=w80) -> ("TRANSLATION3D"=w75:T3)  [unwired: 8 in]
  n58 = call <vilib>:"Rotation3d_Create_RollPitchYaw.vi"("Yaw"=w76, "Pitch"=w77, "Roll"=w78) -> ("Rotation3d"=w74:T4)  [unwired: 8 in]
  n59 = call <vilib>:"Transform3d_Create_Trans3dRot3d.vi"("Rotation3d"=w74, "Translation3d"=w75) -> ("Transform3d"=w4:T8)  [unwired: 9 in]
  n60 = call <vilib>:"Translation3d_Create.vi"("Z"=w69, "Y"=w67, "X"=w68) -> ("TRANSLATION3D"=w63:T3)  [unwired: 8 in]
  n61 = call <vilib>:"Rotation3d_Create_RollPitchYaw.vi"("Yaw"=w64, "Pitch"=w65, "Roll"=w66) -> ("Rotation3d"=w62:T4)  [unwired: 8 in]
  n62 = call <vilib>:"Pose3d_New_Trans3dRot3d.vi"("Rotation3d"=w62, "Translation3d"=w63) -> ("outPose3d"=w7:T2)  [unwired: 9 in]
  n63 = call <vilib>:"PhotonPoseEstimator_New.vi"("RobotToCamera"=w4, "Camera"=w3, "Strategy"=w2, "AprilTagFieldLayout"=w6) -> ("PhotonPoseEstimator"=w48:T17)  [unwired: 7 in]
  n64 = call <vilib>:"PhotonPoseEstimator_PackConfig.vi"("RobotToCamera"=w4, "HighestAmbiguity"=w1, "PirmaryStrategy"=w2, "Camera"=w3) -> ("PoseEstimator_Configuration"=w5:T19)  [unwired: 7 in]
  n65 = call <vilib>:"PhotonPoseEstimator_SetHighestAmbiguity.vi"("HighestAmbiguity"=w1, "PhotonPoseEstimator"=w48) -> ("out PhotonPoseEstimator"=w47:T17)  [unwired: 9 in]
  n66 = call <vilib>:"PhotonPoseEstimator_SetReferencePose.vi"("ReferencePose"=w7, "PhotonPoseEstimator"=w47) -> ("out PhotonPoseEstimator"=w46:T17)  [unwired: 9 in]
  n67 = call <vilib>:"PhotonPoseEstimator_Update_PipeResult.vi"("Has Results"=w8, "PipelineResult"=w9, "PhotonPoseEstimator"=w46) -> ("Pos Found"=→"Pos Found":bool, "PhotonEstimatedRobotPose"=w61:T1)  [unwired: 6 in, 1 out]
  "PhotonEstimatedRobotPose" <- w61
  n68 = call <vilib>:"PhotonPoseEstimator_Update_ClosestToReferencePose.vi"("Has Results"=w8, "PipelineResult"=w9, "PhotonPoseEstimator"=w46) -> ("PhotonEstimatedRobotPose"=w29:T1)  [unwired: 6 in, 2 out]
  n69 = call <vilib>:"PhotonPoseEstimator_Execute_ClosestToReferencePose.vi"("Configuration"=w5, "AprilTagFieldLayout"=w6, "ReferencePose"=w7, "PIpeline Has \nNew Results"=w8, "PipelineResult"=w9) -> ("PhotonEstimatedRobotPose"=w10:T1)  [unwired: 1 in, 5 out]
  n70 = Unbundle By Name(w61) -> ("TimeStamp_Seconds"=w70:dbl, "EstimatedPose.Translation3d.X"=w84:dbl, "EstimatedPose.Translation3d.Y"=w83:dbl, "EstimatedPose.Translation3d.Z"=w82:dbl)
  n71 = Unbundle By Name(w29) -> ("TimeStamp_Seconds"=w30:dbl, "EstimatedPose.Translation3d.X"=w36:dbl, "EstimatedPose.Translation3d.Y"=w35:dbl, "EstimatedPose.Translation3d.Z"=w34:dbl)
  n72 = Unbundle By Name(w10) -> ("TimeStamp_Seconds"=w12:dbl, "EstimatedPose.Translation3d.X"=w18:dbl, "EstimatedPose.Translation3d.Y"=w17:dbl, "EstimatedPose.Translation3d.Z"=w16:dbl)
  n73 = call <vilib>:"Util_ApproxEquals.vi"("Tolerance"=0.01, "Value 2"=17.0, "Value 1"=w70) -> ("ApproxEquals"=w71:bool)  [unwired: 8 in]
  n74 = call <vilib>:"Util_ApproxEquals.vi"("Tolerance"=0.01, "Value 2"=1.1, "Value 1"=w83) -> ("ApproxEquals"=w86:bool)  [unwired: 8 in]
  n75 = call <vilib>:"Util_ApproxEquals.vi"("Tolerance"=0.01, "Value 2"=1.0, "Value 1"=w84) -> ("ApproxEquals"=w249:bool)  [unwired: 8 in]
  n76 = call <vilib>:"Util_ApproxEquals.vi"("Tolerance"=0.01, "Value 2"=17.0, "Value 1"=w30) -> ("ApproxEquals"=w31:bool)  [unwired: 8 in]
  n77 = call <vilib>:"Util_ApproxEquals.vi"("Tolerance"=0.01, "Value 2"=0.9, "Value 1"=w82) -> ("ApproxEquals"=w85:bool)  [unwired: 8 in]
  n78 = call <vilib>:"Util_ApproxEquals.vi"("Tolerance"=0.01, "Value 2"=1.1, "Value 1"=w35) -> ("ApproxEquals"=w38:bool)  [unwired: 8 in]
  n79 = call <vilib>:"Util_ApproxEquals.vi"("Tolerance"=0.01, "Value 2"=1.0, "Value 1"=w36) -> ("ApproxEquals"=w43:bool)  [unwired: 8 in]
  n80 = call <vilib>:"Util_ApproxEquals.vi"("Tolerance"=0.01, "Value 2"=0.9, "Value 1"=w34) -> ("ApproxEquals"=w37:bool)  [unwired: 8 in]
  n81 = call <vilib>:"Util_ApproxEquals.vi"("Tolerance"=0.01, "Value 2"=17.0, "Value 1"=w12) -> ("ApproxEquals"=w13:bool)  [unwired: 8 in]
  n82 = call <vilib>:"Util_ApproxEquals.vi"("Tolerance"=0.01, "Value 2"=1.1, "Value 1"=w17) -> ("ApproxEquals"=w20:bool)  [unwired: 8 in]
  n83 = call <vilib>:"Util_ApproxEquals.vi"("Tolerance"=0.01, "Value 2"=1.0, "Value 1"=w18) -> ("ApproxEquals"=w25:bool)  [unwired: 8 in]
  n84 = call <vilib>:"Util_ApproxEquals.vi"("Tolerance"=0.01, "Value 2"=0.9, "Value 1"=w16) -> ("ApproxEquals"=w19:bool)  [unwired: 8 in]
  n85 = Compound Arithmetic op=AND(w71, w249, w86, w85) -> (w247:bool)
  "Test 0 Passed" <- w247
  n86 = Compound Arithmetic op=AND(w31, w43, w38, w37) -> (w28:bool)
  "Test 1 Passed" <- w28
  n87 = Compound Arithmetic op=AND(w13, w25, w20, w19) -> (w11:bool)
  "Test 2 Passed" <- w11
  n88 = Compound Arithmetic op=AND(w247, w28, w11) -> (→"Test Passed":bool)
  "error out" <- "error in (no error)"
